vi "test tool required arguments.vi"(8 "error in (no error)":errorcluster) -> (0 "error out":errorcluster, 3 "body":string)   [LabVIEW 2020, in "MCP Server tests.lvlib"]
doc: "tools/call that leaves out a required input of the tool (one set to Required on the connector pane) is answered with a normal result with isError true and one text item that names the missing arguments in the order of inputSchema.required (Missing required argument(s): ...), so that the model can correct the call. It is not a JSON-RPC error, and the tool is not run. With all required arguments the tool runs. fake_tool_required_input has the required inputs a and b."
uses:
  MCP Server tests.lvlib
  2843e6e7-508a-4314-8b34-edca1324cd47.vi
  1722cc8e-d948-415c-9422-97d44714415d.vi
  4bf96725-8387-4906-b640-b116e14cb2fd.vi
  31daec1a-f8fb-4278-b5db-ae2098a396f1.vi
  <vilib>/JDP Science/JSONtext/Next JSON Value.vi
  <vilib>/JDP Science/JSONtext/String Subset.vi
  <vilib>/JDP Science/JSONtext/Parsing/Advance past next JSON Value (inlined COPY).vi
  <vilib>/JDP Science/JSONtext/Parsing/Advance past whitespace.vi
  <vilib>/JDP Science/JSONtext/Parsing/Advance past String.vi
  <vilib>/JDP Science/JSONtext/Parsing/Advance past Number.vi
  <vilib>/JDP Science/JSONtext/Parsing/Advance past Line Ending.vi
  <vilib>/JDP Science/JSONtext/Parsing/Parse Full Path or Item Name.vi
  <vilib>/JDP Science/JSONtext/Parsing/Advance past Array.vi
  <vilib>/JDP Science/JSONtext/Parsing/Advance past Object.vi
  <vilib>/JDP Science/JSONtext/support/Error Cluster From Code.vi
  <vilib>/JDP Science/JSONtext/Offset/Find Item Locations by Path.vi
  <vilib>/JDP Science/JSONtext/JSON text to Variant.vi
  <vilib>/JDP Science/JSONtext/LVClass Serializer/JSONtext LVClass Serializer.lvclass
  <vilib>/addons/_JKI Toolkits/Caraya/classes/Test/Test.lvclass
  <vilib>/JDP Science/JSONtext/JSONtext.lvlib
  <vilib>/addons/_JKI Toolkits/Caraya/classes/Assert/Assert.lvclass
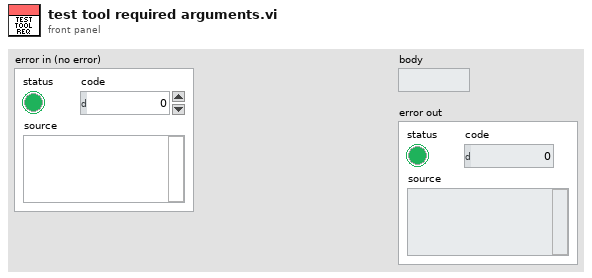
[diagram p1: front panel]
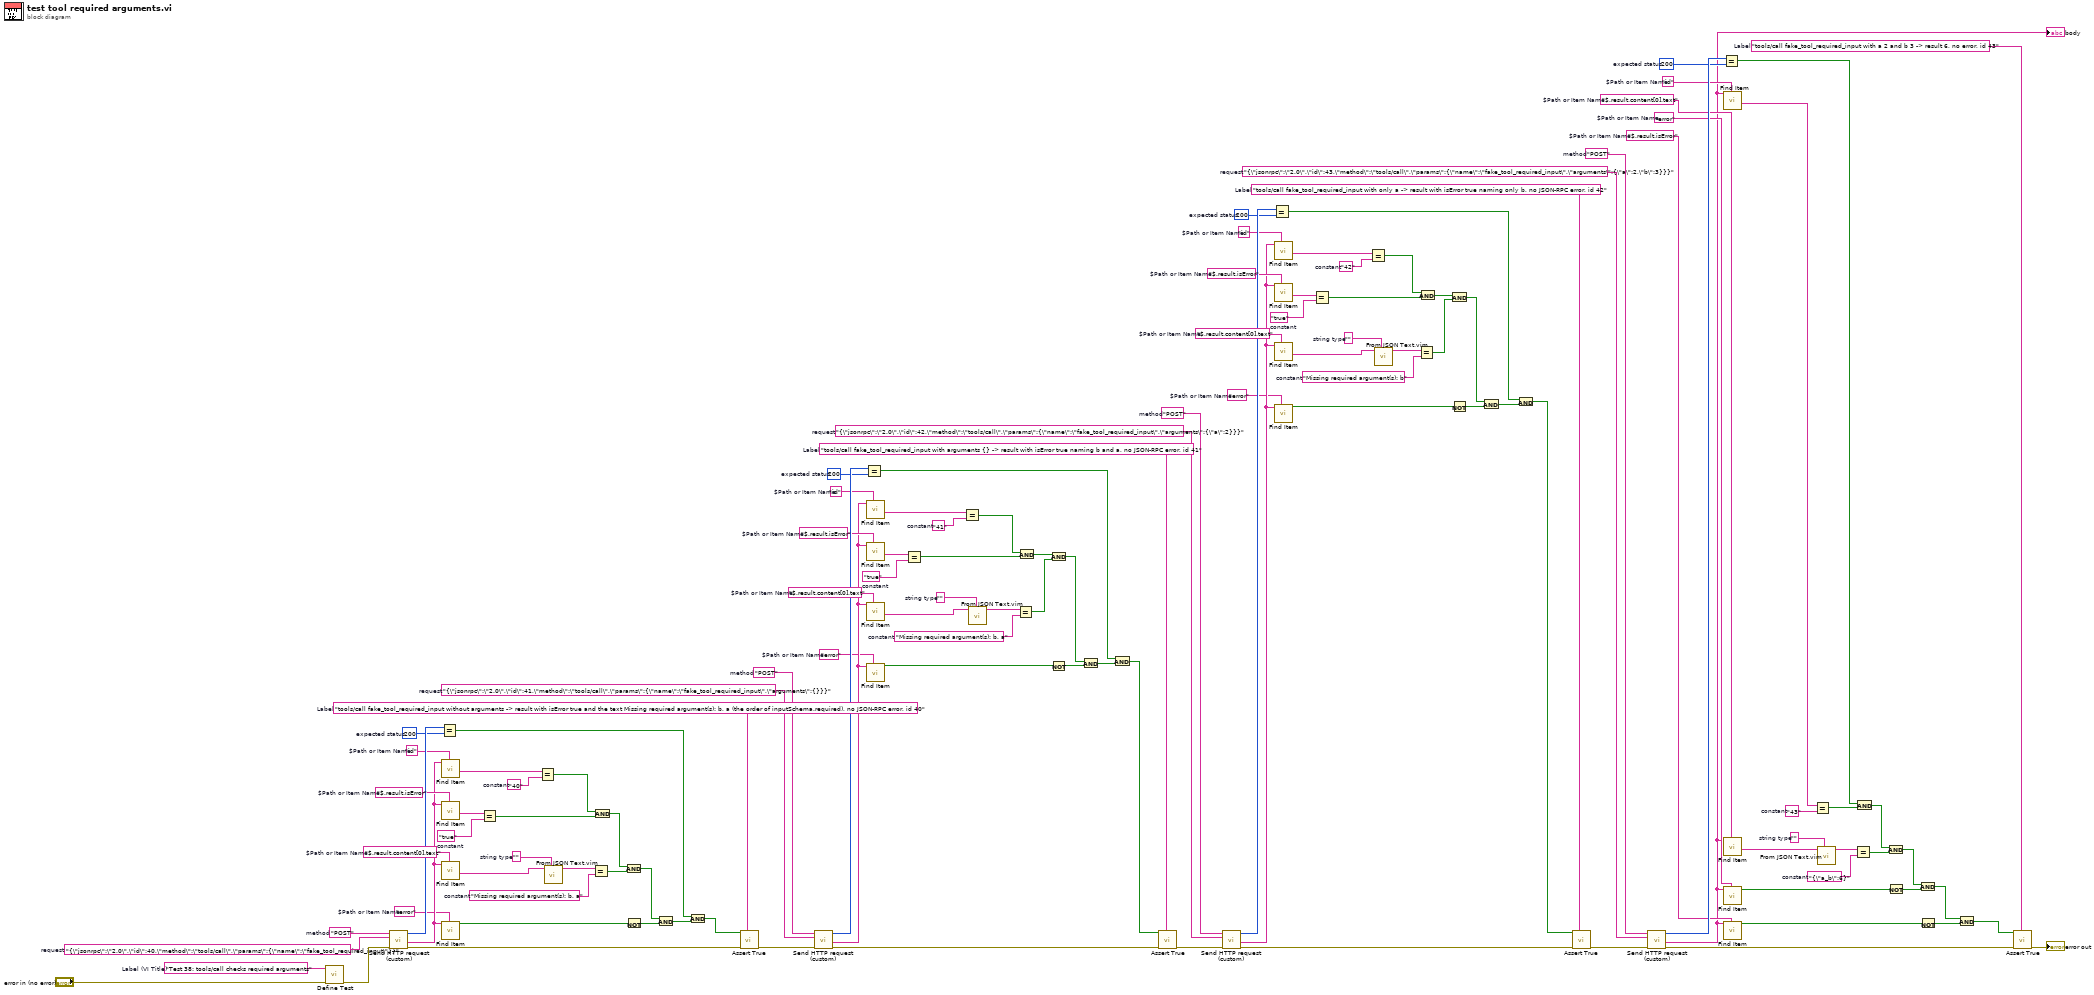
[diagram p0: block diagram]
diagram:
  w3 = "tools/call fake_tool_required_input with a 2 and b 3 -> result 6, no error, id 43"  # Label
  w16 = "{\"a_b\":6}"  # constant
  w18 = ""  # string type
  w20 = "43"  # constant
  w22 = "$.result.isError"  # $Path or Item Name
  w23 = "error"  # $Path or Item Name
  w24 = "$.result.content[0].text"  # $Path or Item Name
  w25 = "id"  # $Path or Item Name
  w26 = 200  # expected status
  w29 = "{\"jsonrpc\":\"2.0\",\"id\":43,\"method\":\"tools/call\",\"params\":{\"name\":\"fake_tool_required_input\",\"arguments\":{\"a\":2,\"b\":3}}}"  # request
  w30 = "POST"  # method
  w31 = "tools/call fake_tool_required_input with only a -> result with isError true naming only b, no JSON-RPC error, id 42"  # Label
  w43 = "Missing required argument(s): b"  # constant
  w45 = ""  # string type
  w47 = "true"  # constant
  w49 = "42"  # constant
  w51 = "error"  # $Path or Item Name
  w53 = "$.result.content[0].text"  # $Path or Item Name
  w54 = "$.result.isError"  # $Path or Item Name
  w55 = "id"  # $Path or Item Name
  w56 = 200  # expected status
  w59 = "{\"jsonrpc\":\"2.0\",\"id\":42,\"method\":\"tools/call\",\"params\":{\"name\":\"fake_tool_required_input\",\"arguments\":{\"a\":2}}}"  # request
  w60 = "POST"  # method
  w61 = "tools/call fake_tool_required_input with arguments {} -> result with isError true naming b and a, no JSON-RPC error, id 41"  # Label
  w73 = "Missing required argument(s): b, a"  # constant
  w75 = ""  # string type
  w77 = "true"  # constant
  w79 = "41"  # constant
  w81 = "error"  # $Path or Item Name
  w83 = "$.result.content[0].text"  # $Path or Item Name
  w84 = "$.result.isError"  # $Path or Item Name
  w85 = "id"  # $Path or Item Name
  w86 = 200  # expected status
  w89 = "{\"jsonrpc\":\"2.0\",\"id\":41,\"method\":\"tools/call\",\"params\":{\"name\":\"fake_tool_required_input\",\"arguments\":{}}}"  # request
  w90 = "POST"  # method
  w91 = "tools/call fake_tool_required_input without arguments -> result with isError true and the text Missing required argument(s): b, a (the order of inputSchema.required), no JSON-RPC error, id 40"  # Label
  w103 = "Missing required argument(s): b, a"  # constant
  w105 = ""  # string type
  w107 = "true"  # constant
  w109 = "40"  # constant
  w111 = "error"  # $Path or Item Name
  w113 = "$.result.content[0].text"  # $Path or Item Name
  w114 = "$.result.isError"  # $Path or Item Name
  w115 = "id"  # $Path or Item Name
  w116 = 200  # expected status
  w119 = "{\"jsonrpc\":\"2.0\",\"id\":40,\"method\":\"tools/call\",\"params\":{\"name\":\"fake_tool_required_input\"}}"  # request
  w120 = "POST"  # method
  w122 = "Test 38: tools/call checks required arguments"  # Label (VI Title)
  n1 = call <vilib>:"Define Test.vi"("error in (no error)"="error in (no error)", "Label (VI Title)"=w122) -> ("error out"=w118:errorcluster)  [unwired: 8 in, 1 out]
  n2 = call "Send HTTP request (custom).vi"("error in (no error)"=w118, "request"=w119, "method"=w120) -> ("error out"=w92:errorcluster, "response"=w112:string, "status code"=w117:i32)  [unwired: 5 in, 1 out]
  n3 = Equal?(x=w117, y=w116) -> (x = y?=w95:bool)
  n4 = call <vilib>:"Find Item.vi"("$Path or Item Name"=w115, "JSON"=w112) -> ("<JSON>"=w110:string)  [unwired: 6 in, 3 out]
  n5 = call <vilib>:"Find Item.vi"("$Path or Item Name"=w114, "JSON"=w112) -> ("<JSON>"=w108:string)  [unwired: 6 in, 3 out]
  n6 = call <vilib>:"Find Item.vi"("$Path or Item Name"=w113, "JSON"=w112) -> ("<JSON>"=w106:string)  [unwired: 6 in, 3 out]
  n7 = call <vilib>:"Find Item.vi"("$Path or Item Name"=w111, "JSON"=w112) -> ("Found"=w102:bool)  [unwired: 6 in, 3 out]
  n8 = Equal?(x=w108, y=w107) -> (x = y?=w100:bool)
  n9 = Equal?(x=w110, y=w109) -> (x = y?=w101:bool)
  n10 = call "From JSON Text.vim"("Data Type and Default Value"=w105, "JSON"=w106) -> ("Data out"=w104:string)  [unwired: 8 in, 1 out]
  n11 = Equal?(x=w104, y=w103) -> (x = y?=w98:bool)
  n12 = And(x=w101, y=w100) -> (x .and. y?=w99:bool)
  n13 = And(x=w99, y=w98) -> (x .and. y?=w97:bool)
  n14 = Not(x=w102) -> (.not. x?=w96:bool)
  n15 = And(x=w97, y=w96) -> (x .and. y?=w94:bool)
  n16 = And(x=w95, y=w94) -> (x .and. y?=w93:bool)
  n17 = call <vilib>:"Assert True.vi"("Label"=w91, "error in (no error)"=w92, "True?"=w93) -> ("error out"=w88:errorcluster)  [unwired: 7 in, 1 out]
  n18 = call "Send HTTP request (custom).vi"("error in (no error)"=w88, "request"=w89, "method"=w90) -> ("error out"=w62:errorcluster, "response"=w82:string, "status code"=w87:i32)  [unwired: 5 in, 1 out]
  n19 = Equal?(x=w87, y=w86) -> (x = y?=w65:bool)
  n20 = call <vilib>:"Find Item.vi"("$Path or Item Name"=w85, "JSON"=w82) -> ("<JSON>"=w80:string)  [unwired: 6 in, 3 out]
  n21 = call <vilib>:"Find Item.vi"("$Path or Item Name"=w84, "JSON"=w82) -> ("<JSON>"=w78:string)  [unwired: 6 in, 3 out]
  n22 = call <vilib>:"Find Item.vi"("$Path or Item Name"=w83, "JSON"=w82) -> ("<JSON>"=w76:string)  [unwired: 6 in, 3 out]
  n23 = call <vilib>:"Find Item.vi"("$Path or Item Name"=w81, "JSON"=w82) -> ("Found"=w72:bool)  [unwired: 6 in, 3 out]
  n24 = Equal?(x=w78, y=w77) -> (x = y?=w70:bool)
  n25 = Equal?(x=w80, y=w79) -> (x = y?=w71:bool)
  n26 = call "From JSON Text.vim"("Data Type and Default Value"=w75, "JSON"=w76) -> ("Data out"=w74:string)  [unwired: 8 in, 1 out]
  n27 = Equal?(x=w74, y=w73) -> (x = y?=w68:bool)
  n28 = And(x=w71, y=w70) -> (x .and. y?=w69:bool)
  n29 = And(x=w69, y=w68) -> (x .and. y?=w67:bool)
  n30 = Not(x=w72) -> (.not. x?=w66:bool)
  n31 = And(x=w67, y=w66) -> (x .and. y?=w64:bool)
  n32 = And(x=w65, y=w64) -> (x .and. y?=w63:bool)
  n33 = call <vilib>:"Assert True.vi"("Label"=w61, "error in (no error)"=w62, "True?"=w63) -> ("error out"=w58:errorcluster)  [unwired: 7 in, 1 out]
  n34 = call "Send HTTP request (custom).vi"("error in (no error)"=w58, "request"=w59, "method"=w60) -> ("error out"=w32:errorcluster, "response"=w52:string, "status code"=w57:i32)  [unwired: 5 in, 1 out]
  n35 = Equal?(x=w57, y=w56) -> (x = y?=w35:bool)
  n36 = call <vilib>:"Find Item.vi"("$Path or Item Name"=w55, "JSON"=w52) -> ("<JSON>"=w50:string)  [unwired: 6 in, 3 out]
  n37 = call <vilib>:"Find Item.vi"("$Path or Item Name"=w54, "JSON"=w52) -> ("<JSON>"=w48:string)  [unwired: 6 in, 3 out]
  n38 = call <vilib>:"Find Item.vi"("$Path or Item Name"=w53, "JSON"=w52) -> ("<JSON>"=w46:string)  [unwired: 6 in, 3 out]
  n39 = call <vilib>:"Find Item.vi"("$Path or Item Name"=w51, "JSON"=w52) -> ("Found"=w42:bool)  [unwired: 6 in, 3 out]
  n40 = Equal?(x=w48, y=w47) -> (x = y?=w40:bool)
  n41 = Equal?(x=w50, y=w49) -> (x = y?=w41:bool)
  n42 = call "From JSON Text.vim"("Data Type and Default Value"=w45, "JSON"=w46) -> ("Data out"=w44:string)  [unwired: 8 in, 1 out]
  n43 = Equal?(x=w44, y=w43) -> (x = y?=w38:bool)
  n44 = And(x=w41, y=w40) -> (x .and. y?=w39:bool)
  n45 = And(x=w39, y=w38) -> (x .and. y?=w37:bool)
  n46 = Not(x=w42) -> (.not. x?=w36:bool)
  n47 = And(x=w37, y=w36) -> (x .and. y?=w34:bool)
  n48 = And(x=w35, y=w34) -> (x .and. y?=w33:bool)
  n49 = call <vilib>:"Assert True.vi"("Label"=w31, "error in (no error)"=w32, "True?"=w33) -> ("error out"=w28:errorcluster)  [unwired: 7 in, 1 out]
  n50 = call "Send HTTP request (custom).vi"("error in (no error)"=w28, "request"=w29, "method"=w30) -> ("error out"=w4:errorcluster, "response"=w2:string, "status code"=w27:i32)  [unwired: 5 in, 1 out]
  "body" <- w2
  n51 = Equal?(x=w27, y=w26) -> (x = y?=w13:bool)
  n52 = call <vilib>:"Find Item.vi"("$Path or Item Name"=w25, "JSON"=w2) -> ("<JSON>"=w21:string)  [unwired: 6 in, 3 out]
  n53 = call <vilib>:"Find Item.vi"("$Path or Item Name"=w24, "JSON"=w2) -> ("<JSON>"=w19:string)  [unwired: 6 in, 3 out]
  n54 = call <vilib>:"Find Item.vi"("$Path or Item Name"=w23, "JSON"=w2) -> ("Found"=w15:bool)  [unwired: 6 in, 3 out]
  n55 = call <vilib>:"Find Item.vi"("$Path or Item Name"=w22, "JSON"=w2) -> ("Found"=w14:bool)  [unwired: 6 in, 3 out]
  n56 = Equal?(x=w21, y=w20) -> (x = y?=w12:bool)
  n57 = call "From JSON Text.vim"("Data Type and Default Value"=w18, "JSON"=w19) -> ("Data out"=w17:string)  [unwired: 8 in, 1 out]
  n58 = Equal?(x=w17, y=w16) -> (x = y?=w10:bool)
  n59 = And(x=w13, y=w12) -> (x .and. y?=w11:bool)
  n60 = And(x=w11, y=w10) -> (x .and. y?=w9:bool)
  n61 = Not(x=w15) -> (.not. x?=w8:bool)
  n62 = And(x=w9, y=w8) -> (x .and. y?=w7:bool)
  n63 = Not(x=w14) -> (.not. x?=w6:bool)
  n64 = And(x=w7, y=w6) -> (x .and. y?=w5:bool)
  n65 = call <vilib>:"Assert True.vi"("Label"=w3, "error in (no error)"=w4, "True?"=w5) -> ("error out"=→"error out":errorcluster)  [unwired: 7 in, 1 out]
